vi "Configure Session.vi"(8 "error in":errorcluster, 11 "Plugin in":refnum<class "Modbus.lvclass">) -> (0 "error out":errorcluster, 3 "Plugin out":refnum<class "Modbus.lvclass">)   [LabVIEW 2026, in "Modbus.lvlib" / "Modbus.lvclass"]
uses:
  Modbus.lvclass
  C:/Program Files/National Instruments/LabVIEW 2026/vi.lib/FlexLogger/SDK/PluginSDK.lvlibp/PEFClasses/SDK/Plugin/Plugin.lvclass
  <vilib>/FlexLogger/SDK/PluginSDK.lvlibp/PEFClasses/SDK/Plugin/Plugin.lvclass
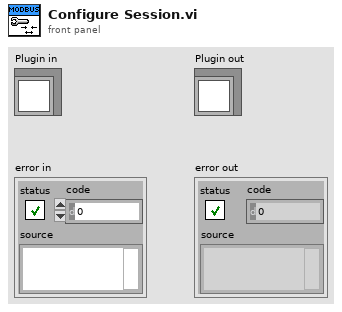
[diagram p1: front panel]
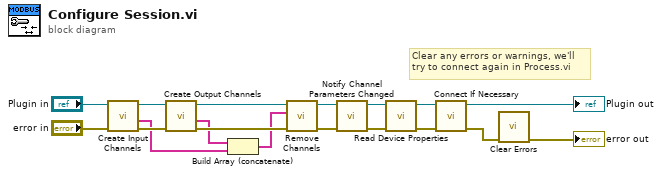
[diagram p0: block diagram]
diagram:
  # "Clear any errors or warnings, we'll\ntry to connect again in Process.vi"
  n1 = call "Create Input Channels.vi"("error in (no error)"="error in", "Modbus in"="Plugin in") -> ("error out"=w14:errorcluster, "Channels to remove"=w12:string[], "Modbus out"=w16:refnum<class "Modbus.lvclass">)  [unwired: 7 in]
  n2 = call "Create Output Channels.vi"("error in (no error)"=w14, "Modbus in"=w16) -> ("error out"=w13:errorcluster, "Channels to remove"=w11:string[], "Modbus out"=w15:refnum<class "Modbus.lvclass">)  [unwired: 7 in]
  n3 = Build Array (concatenate)(w11, w12) -> (w10:string[])
  n4 = call-dynamic "Remove Channels.vi"("error in (no error)"=w13, "Unique Channel Identifiers to Delete"=w10, "Plugin in"=w15) -> ("error out"=w7:errorcluster, "Plugin out"=w8:refnum<class "Modbus.lvclass">)  [unwired: 7 in]
  n5 = call <vilib>:"Notify Channel Parameters Changed.vi"("error in (no error)"=w7, "Plugin in"=w8) -> ("error out"=w5:errorcluster, "Plugin out"=w6:refnum<class "Modbus.lvclass">)  [unwired: 8 in]
  n6 = call "Read Device Properties.vi"("error in (no error)"=w5, "Modbus in"=w6) -> ("error out"=w9:errorcluster, "Modbus out"=w4:refnum<class "Modbus.lvclass">)  [unwired: 8 in]
  n7 = call "Connect If Necessary.vi"("error in (no error)"=w9, "Plugin in"=w4) -> ("error out"=w3:errorcluster, "Plugin out"=→"Plugin out":refnum<class "Modbus.lvclass">)  [unwired: 8 in]
  n8 = call <vilib>:"Clear Errors.vi"("error in (no error)"=w3) -> ("error out"=→"error out":errorcluster)  [unwired: 5 in, 1 out]
